vi "Set Datatype.vi"(8 "error in":errorcluster, 10 "Datatype":T1, 11 "IElement in":refnum<class "IElement.lvclass">) -> (0 "error out":errorcluster, 3 "IElement out":refnum<class "IElement.lvclass">)   [LabVIEW 2026, in "IElement.lvclass"]
doc: "Set Datatype."
uses:
  IElement.lvclass
  Type Definitions/Data types--enum.ctl
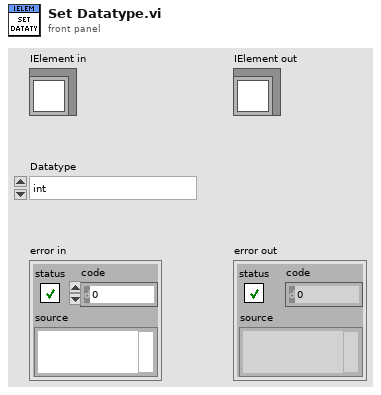
[diagram p1: front panel]
types:
  T1 = typedef "Data types--enum.ctl" = enum16{"int", "float", "bool", "str", "complex", "TypedDict", "np.bool_", "np.int8", "np.int16", "np.int32", "np.int64", "np.uint8", "np.uint16", "np.uint32", "np.uint64", "np.float32", "np.float64", "np.complex64", "np.complex128", "np.str_"}
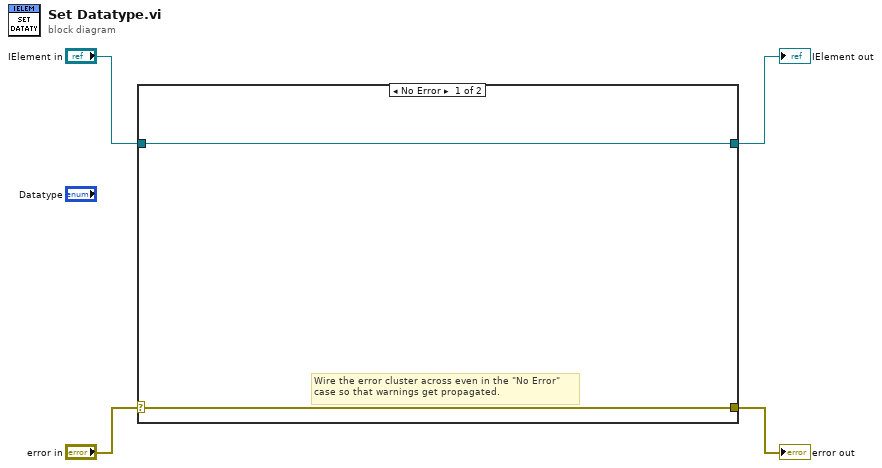
[diagram p0: block diagram]
diagram:
  n1 = case shown="No Error" "error in" {
    selector: "error in" -> [w6 w8]
    tunnel: [w6 w8] -> w3
    tunnel: [w5 w7] -> w1
    tunnel: "IElement in" -> [w5 w7]
    frame No Error {
      # "Wire the error cluster across even in the \"No Error\"\ncase so that warnings get propagated."
    }
    frame Error {
    }
  }
  "error out" <- w3
  "IElement out" <- w1
